vi "Cycle_Begin.vi"(8 "error in (no error)":errorcluster={"status"=FALSE, "code"=0, "source"="\"\""}, 11 "Counter set and cycle policy":string) -> (0 "error out":errorcluster={"status"=FALSE, "code"=0, "source"="\"\""}, 2 "status ok":bool, 3 "New cycle identity":string)   [LabVIEW 2026]
doc: "INTENT: Begin group/test repetition. LOGIC: Assign monotonic attempt ID, advance started count and open result scope."
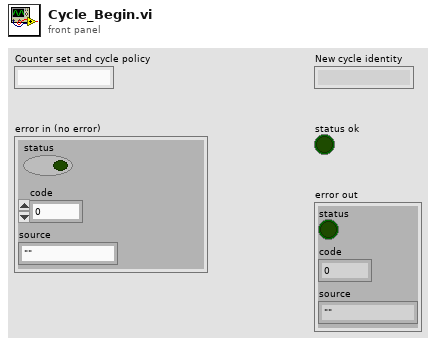
[diagram p1: front panel]
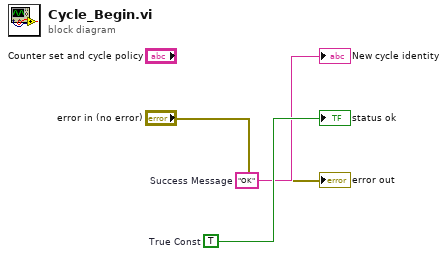
[diagram p0: block diagram]
diagram:
  w3 = TRUE  # True Const
  w2 = "OK"  # Success Message
  "New cycle identity" <- w2
  "status ok" <- w3
  "error out" <- "error in (no error)"
